vi "VIH Project - Get Default Template File Path.vi"(10 "Template Type":enum16{"menu", "VI", "PolyVI"}(ring), 11 "Path":path) -> (3 "Path out":path)   [LabVIEW 2014]
doc: "::: VI Helpeks :::\nCopyright (c) 2000-2026 Konstantin Shifershteyn. All rights reserved."
panel:
  # "VI Helpeks\nCopyright (c) 2012-2026 Konstantin Shifershteyn"
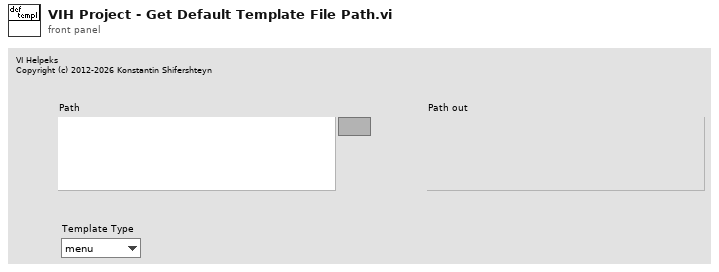
[diagram p1: front panel]
types:
  T1 = typedef "VIH HelpGen Typedef - Cluster - Group Rule.ctl" = cluster{"Source Root Dir":path, "Build Root Dir":path, "BuildHelp":T2, "Source Paths":T3, "Target Paths":T4, "VIDscrMode":T5, "MenuDscrMode":T5, "MenuItemIcons":T2, "Control Rules":T6[], "Flags":T8, "Ctl_DscrMode":T5, "Ctl_ClustMembers":T2, "Ctl_EnumValues":T2, "%Comments":string, "PVIIDscrMode":T5, "VIDetailsMode":T5, "ProductInfoMode":T2, "ProductInfoText":string}
  T2 = typedef "VIH HelpGen Typedef - Enum - Default,Enable,Disable.ctl" = enum16{"Default", "Enable", "Disable"}
  T3 = typedef "VIH HelpGen Typedef - Cluster - Group Rule - Source Paths.ctl" = cluster{"CSS Files":path[], "JS Files":path[], "VI Template":path, "Menu Template":path, "PolyVI Template":path}
  T4 = typedef "VIH HelpGen Typedef - Cluster - Group Rule - Target Paths.ctl" = cluster{"HTML Dir":path, "Image Dir":path, "CSS Dir":path, "JS Dir":path}
  T5 = typedef "VIH HelpGen Typedef - Enum - Description Mode.ctl" = enum16{"Default", "Description", "Description1", "Description2", "Custom", "None"}
  T6 = typedef "VIH HelpGen Typedef - Cluster - Control Rule.ctl" = cluster{"CtrlID":string, "CustomRule":bool, "DscrMode":T5, "Description":string, "ClusterMembers":T2, "EnumValues":T2, "EnumValDscr":T7[], "CustomName":string}
  T7 = typedef "VIH HelpGen Typedef - Cluster - Enum Value Info.ctl" = cluster{"Value":ext, "String":string, "Description":string}
  T8 = typedef "VIH HelpGen Typedef - Cluster - Group Rule - Flags.ctl" = cluster{"Override CSS Files":bool, "Override JS Files":bool, "Override Ctl Rules":bool}
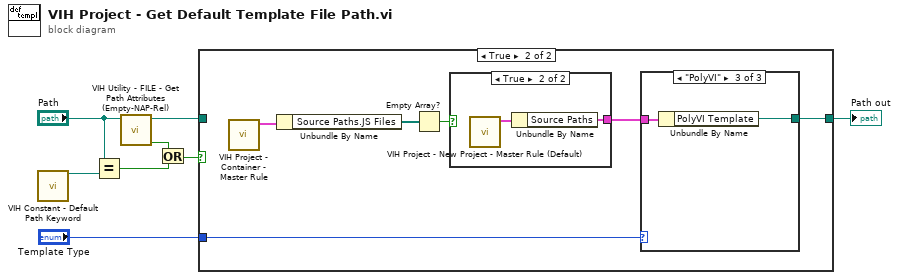
[diagram p0: block diagram]
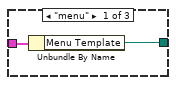
[diagram p3: hidden frame]
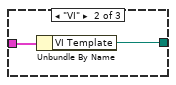
[diagram p4: hidden frame]
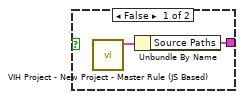
[diagram p5: hidden frame]
diagram:
  n1 = call "VIH Constant - Default Path Keyword.vi"() -> ("<default> path"=w4:path)  [unwired: 11 in]
  n2 = Equal?(x="Path", y=w4) -> (x = y?=w3:bool)
  n3 = call "VIH Utility - FILE - Get Path Attributes (Empty-NAP-Rel).vi"("Path"="Path") -> ("Not A Path or Empty path"=w2:bool, "dup Path"=w6:path)  [unwired: 6 in, 3 out]
  n4 = Or(x=w2, y=w3) -> (x .or. y?=w1:bool)
  n5 = case shown="True" w1 {
    tunnel: "Template Type" -> [_ w12]
    tunnel: [w9 w10] -> w7
    tunnel: w6 -> [w9 _]
    frame False {
    }
    frame True {
      n6 = call "VIH Project - Container - Master Rule.vi"() -> ("Rule out"=w15:T1)  [unwired: 11 in]
      n7 = Unbundle By Name(w15) -> ("Source Paths.JS Files"=w14:path[])
      n8 = Empty Array?(array=w14) -> (empty?=w13:bool)
      n9 = case shown="True" w13 {
        tunnel: [w23 w24] -> w11
        frame False {
          n10 = call "VIH Project - New Project - Master Rule (JS Based).vi"() -> ("Master Rule"=w22:T1)  [unwired: 10 in, 1 out]
          n11 = Unbundle By Name(w22) -> ("Source Paths"=w23:T3)
        }
        frame True {
          n12 = call "VIH Project - New Project - Master Rule (Default).vi"() -> ("Master Rule"=w25:T1)  [unwired: 10 in, 1 out]
          n13 = Unbundle By Name(w25) -> ("Source Paths"=w24:T3)
        }
      }
      n14 = case shown="\"PolyVI\"" w12 {
        tunnel: w11 -> [w17 w19 w21]
        tunnel: [w16 w18 w20] -> w10
        frame "menu" {
          n15 = Unbundle By Name(w17) -> ("Menu Template"=w16:path)
        }
        frame "VI" {
          n16 = Unbundle By Name(w19) -> ("VI Template"=w18:path)
        }
        frame "PolyVI" {
          n17 = Unbundle By Name(w21) -> ("PolyVI Template"=w20:path)
        }
      }
    }
  }
  "Path out" <- w7
